vi "PicoScope6000GetStreamingValues.vi"(8 "error in":errorcluster, 11 "handle in":i16) -> (0 "error out":errorcluster, 1 "Trigger":cluster{bool, "triggeredAt":u32}, 2 "Start Index":u32, 3 "handle out":i16, 4 "Number of Samples":u32, 5 "ready":i16, 6 "Auto Stopped":bool)   [LabVIEW 2009]
doc: "This VI is used in streaming mode to get the latest values from the driver. It should be called in a loop after the oscilloscope has been set up using PicoScope6000Settings.vi and streaming has been started by calling PicoScope4000StartStreaming.vi. The VI outputs the number of samples available and the start index of these samples in the array output by PicoScope6000StartStreaming.vi."
uses:
  ps6000Wrap.dll
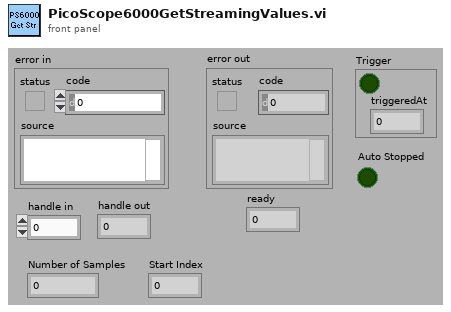
[diagram p1: front panel]
types:
  T1 = cluster{"status":bool, "code":u32, "source":string}
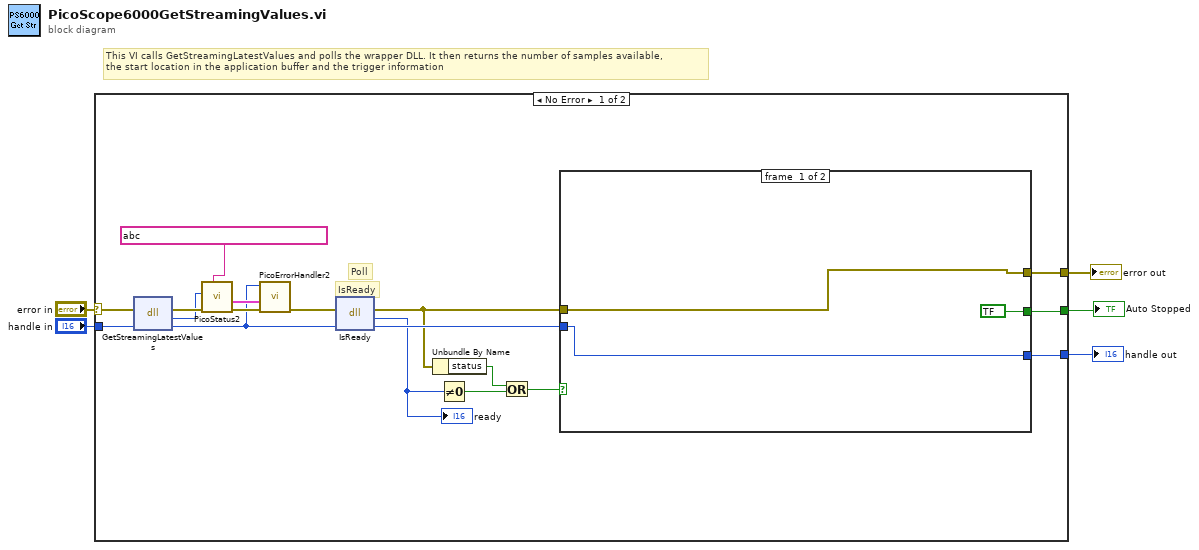
[diagram p0: block diagram]
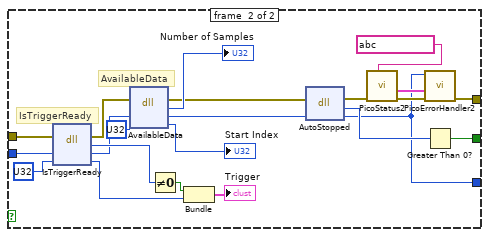
[diagram p2: hidden frame]
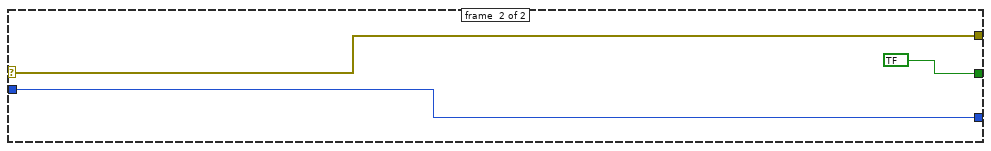
[diagram p3: hidden frame]
diagram:
  # "This VI calls GetStreamingLatestValues and polls the wrapper DLL. It then returns the number of samples available, \nthe start location in the application buffer and the trigger information"
  n1 = case shown="No Error" "error in" {
    selector: "error in" -> [w21 w51]
    tunnel: [w23 w51] -> w4
    tunnel: "handle in" -> [w22 w50]
    tunnel: [w17 w50] -> w2
    tunnel: [w18 bool ?] -> w1
    frame #0 {
      # "Poll"
      # "IsReady"
      n2 = dll-call lib="ps6000wrap.dll" fn="GetStreamingLatestValues" ("PS5000.dll:_ps5000SetDataBuffer@16")(error in=w21, "handle"=w22) -> (error out=w10:errorcluster, "PICO_STATUS"=w6:u32, "handle"=w8:i16)  [unwired: 2 in, 1 out]
      n3 = call "PicoStatus2.vi"("PICO source"=string ? ("source"), "Error in"=w10, "PICO STATUS"=w6) -> ("error out"=w12:errorcluster, "PICO_STATUS out"=w11:T1)  [unwired: 5 in]
      n4 = call "PicoErrorHandler2.vi"("error in (no error)"=w12, "PICO_STATUS in"=w11, "handle In"=w8) -> ("error out"=w9:errorcluster)  [unwired: 8 in]
      n5 = dll-call lib="ps6000wrap.dll" fn="IsReady" ("PS5000.dll:_ps5000SetDataBuffer@16")(error in=w9, "handle"=w8) -> (error out=w19:errorcluster, "ready"=w15:i16, "handle"=w20:i16)  [unwired: 2 in, 1 out]
      "ready" <- w15
      n6 = Unbundle By Name(w19) -> ("status"=w14:bool)
      n7 = Not Equal To 0?(x=w15) -> (x != 0?=w16:bool)
      n8 = Or(x=w14, y=w16) -> (x .or. y?=w13:bool)
      n9 = case shown="True" w13 {
        tunnel: [w26 w29] -> w23
        tunnel: w20 -> [w25 w47]
        tunnel: w19 -> [w26 w40]
        tunnel: [bool ? w33] -> w18
        tunnel: [w25 w28] -> w17
        frame #0 {
        }
        frame #1 {
          # "AvailableData"
          # "IsTriggerReady"
          n10 = dll-call lib="ps6000wrap.dll" fn="IsTriggerReady" ("PS5000.dll:_ps5000SetDataBuffer@16")(error in=w40, "handle"=w47, "triggeredAt"=u32 ?) -> (error out=w42:errorcluster, "triggered"=w46:i16, "handle"=w41:i16, "triggeredAt"=w44:u32)  [unwired: 2 in, 1 out]
          n11 = dll-call lib="ps6000wrap.dll" fn="AvailableData" ("PS5000.dll:_ps5000Stop@4")(error in=w42, "handle"=w41, "startIndex"=u32 ?) -> (error out=w36:errorcluster, "numSamples"=→"Number of Samples":u32, "handle"=w35:i16, "startIndex"=→"Start Index":u32)  [unwired: 2 in, 1 out]
          n12 = Not Equal To 0?(x=w46) -> (x != 0?=w45:bool)
          n13 = Bundle(w45, "triggeredAt"=w44) -> (→"Trigger":cluster{bool, "triggeredAt":u32})  [unwired: 1 in]
          n14 = dll-call lib="ps6000wrap.dll" fn="AutoStopped"(error in=w36, "handle"=w35) -> (error out=w30:errorcluster, "autoStopped"=w34:i16, "handle"=w28:i16)  [unwired: 2 in, 1 out]
          n15 = call "PicoStatus2.vi"("PICO source"=string ? ("source"), "Error in"=w30) -> ("error out"=w31:errorcluster, "PICO_STATUS out"=w32:T1)  [unwired: 6 in]
          n16 = call "PicoErrorHandler2.vi"("error in (no error)"=w31, "PICO_STATUS in"=w32, "handle In"=w28) -> ("error out"=w29:errorcluster)  [unwired: 8 in]
          n17 = Greater Than 0?(x=w34) -> (x > 0?=w33:bool)
        }
      }
    }
    frame #1 {
    }
  }
  "error out" <- w4
  "handle out" <- w2
  "Auto Stopped" <- w1
